vi "Classify Instrument VIs.vi"(0 "InstrContaining":path[][](array[path]), 5 "DestinationDirectory":path[](array[path]), 11 "error in (no error)":errorcluster) -> (4 "InstrContainingVI[]":path[][](array[path]), 15 "error out":errorcluster)   [LabVIEW 2021, in "Multiple Migrator.lvlib"]
uses:
  Multiple Migrator.lvlib
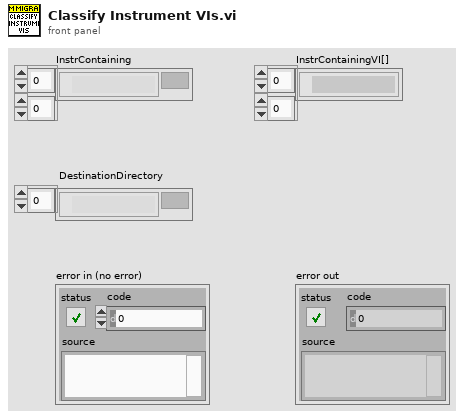
[diagram p1: front panel]
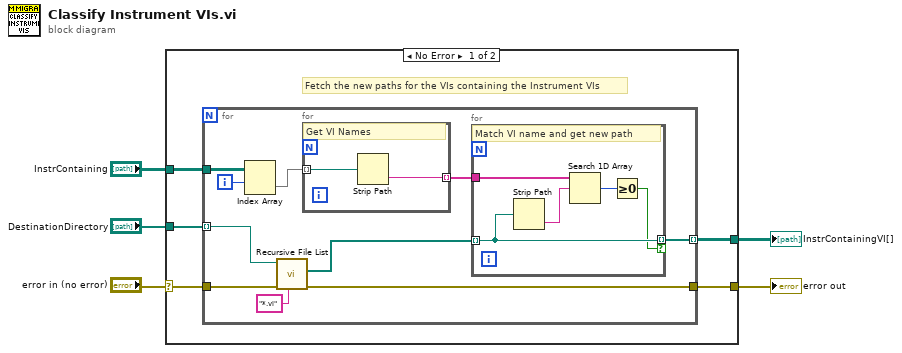
[diagram p0: block diagram]
diagram:
  n1 = case shown="No Error" "error in (no error)" {
    selector: "error in (no error)" -> [w9 w28]
    tunnel: [w7 w28] -> w5
    tunnel: [w10 _] -> w4
    tunnel: "InstrContaining" -> [w8 _]
    tunnel: "DestinationDirectory" -> [w6 _]
    frame No Error {
      # "Fetch the new paths for the VIs containing the Instrument VIs"
      n2 = for {
        tunnel: [w20] -> w10 mode=indexing
        tunnel: w8 -> [w18]
        tunnel: w6 -> [w12] mode=indexing
        tunnel: [w14] -> w7
        tunnel: w9 -> [w13]
        i -> [w17]
        n3 = Index Array(array=w18, index (row)=w17) -> (element=w16:path[])  [unwired: 1 in]
        n4 = call <vilib>:"Recursive File List.vi"("pattern"="*.vi", "error in (no error)"=w13, "Folder Path"=w12) -> ("error out"=w14:errorcluster, "All Files in Dir"=w11:path[])  [unwired: 4 in, 3 out]
        n5 = for {
          tunnel: w16 -> [w22] mode=indexing
          tunnel: [w21] -> w19 mode=indexing
          # "Get VI Names"
          n6 = Strip Path(path=w22) -> (name=w21:string)  [unwired: 1 out]
        }
        n7 = for {
          tunnel: w11 -> [w24] mode=indexing
          tunnel: w19 -> [w27]
          tunnel: [w24] -> w20 mode=indexing if=w23
          # "Match VI name and get new path"
          n8 = Strip Path(path=w24) -> (name=w26:string)  [unwired: 1 out]
          n9 = Search 1D Array(1D array=w27, element=w26) -> (index of element=w25:i32)  [unwired: 1 in]
          n10 = Greater Or Equal To 0?(x=w25) -> (x >= 0?=w23:bool)
        }
      }
    }
    frame Error {
    }
  }
  "error out" <- w5
  "InstrContainingVI[]" <- w4
